vi "VIH HelpGen - Get Control Info.vi"(6 "Ctrl Dscr Params":T5, 8 "error in":errorcluster, 9 "Table Templates":T6, 11 "Ctl Refnum":refnum<vi>) -> (0 "error out":errorcluster, 1 "Image Filename":string, 2 "Ctrl Term Image":T7, 3 "dup Ctl Refnum":refnum<vi>, 4 "Show members":bool, 5 "Ctrl Description":string, 7 "Ctrl Name":string)   [LabVIEW 2014]
doc: "::: VI Helpeks :::\nCopyright (c) 2000-2026 Konstantin Shifershteyn. All rights reserved."
uses:
  <vilib>/picture/picture.llb/imagedata.ctl
  VIH HelpGen Typedef - Table Templates Cluster - VI Help.ctl
  VIH HelpGen Typedef - Cluster - Control Rule.ctl
  VIH HelpGen Typedef - Enum - Description Mode.ctl
  VIH HelpGen Typedef - Enum - Default,Enable,Disable.ctl
  VIH HelpGen Typedef - Cluster - Enum Value Info.ctl
panel:
  # "VI Helpeks\nCopyright (c) 2012-2026 Konstantin Shifershteyn"
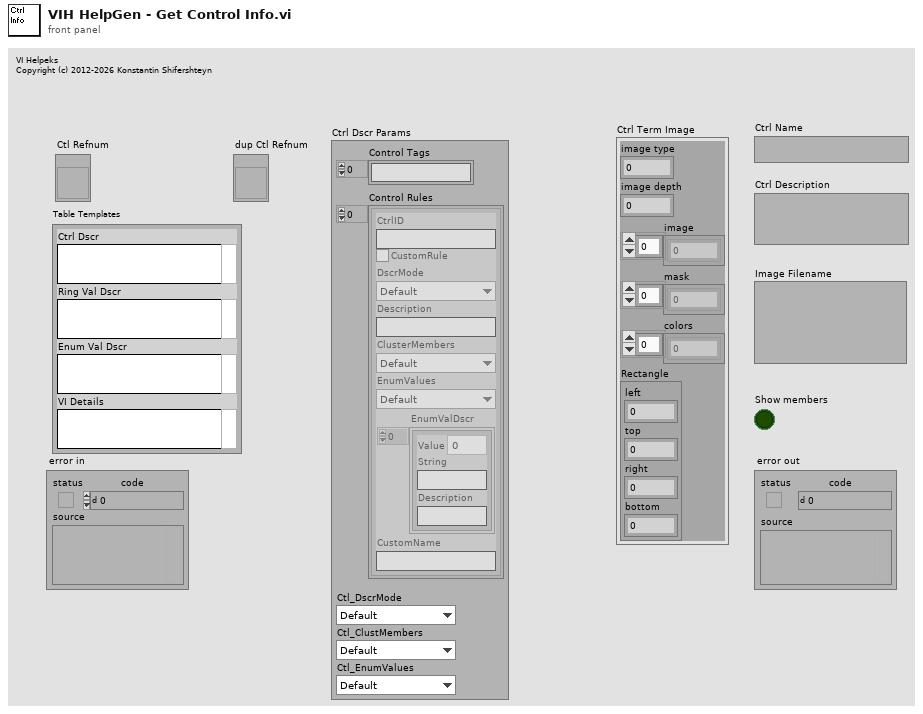
[diagram p1: front panel]
types:
  T1 = typedef "VIH HelpGen Typedef - Cluster - Control Rule.ctl" = cluster{"CtrlID":string, "CustomRule":bool, "DscrMode":T2, "Description":string, "ClusterMembers":T3, "EnumValues":T3, "EnumValDscr":T4[], "CustomName":string}
  T2 = typedef "VIH HelpGen Typedef - Enum - Description Mode.ctl" = enum16{"Default", "Description", "Description1", "Description2", "Custom", "None"}
  T3 = typedef "VIH HelpGen Typedef - Enum - Default,Enable,Disable.ctl" = enum16{"Default", "Enable", "Disable"}
  T4 = typedef "VIH HelpGen Typedef - Cluster - Enum Value Info.ctl" = cluster{"Value":ext, "String":string, "Description":string}
  T5 = cluster{"Control Tags":string[], "Control Rules":T1[], "Ctl_DscrMode":T2, "Ctl_ClustMembers":T3, "Ctl_EnumValues":T3}
  T6 = typedef "VIH HelpGen Typedef - Table Templates Cluster - VI Help.ctl" = cluster{"Ctrl Dscr":string, "Ring Val Dscr":string, "Enum Val Dscr":string, "VI Details":string}
  T7 = typedef "imagedata.ctl" = cluster{"image type":i32, "image depth":i32, "image":u8[], "mask":u8[], "colors":u32[], "Rectangle":cluster{"left":i16, "top":i16, "right":i16, "bottom":i16}}
  T8 = enum32{"not a typedef", "typedef", "strict typedef", "class private data"}
  T9 = enum16{"none", "LV description", "VH minimum", "VH extended"}
  T10 = typedef "LVStringsAndValuesArrayTypeDef.ctl" = cluster{"String":string, "Value":ext}[]
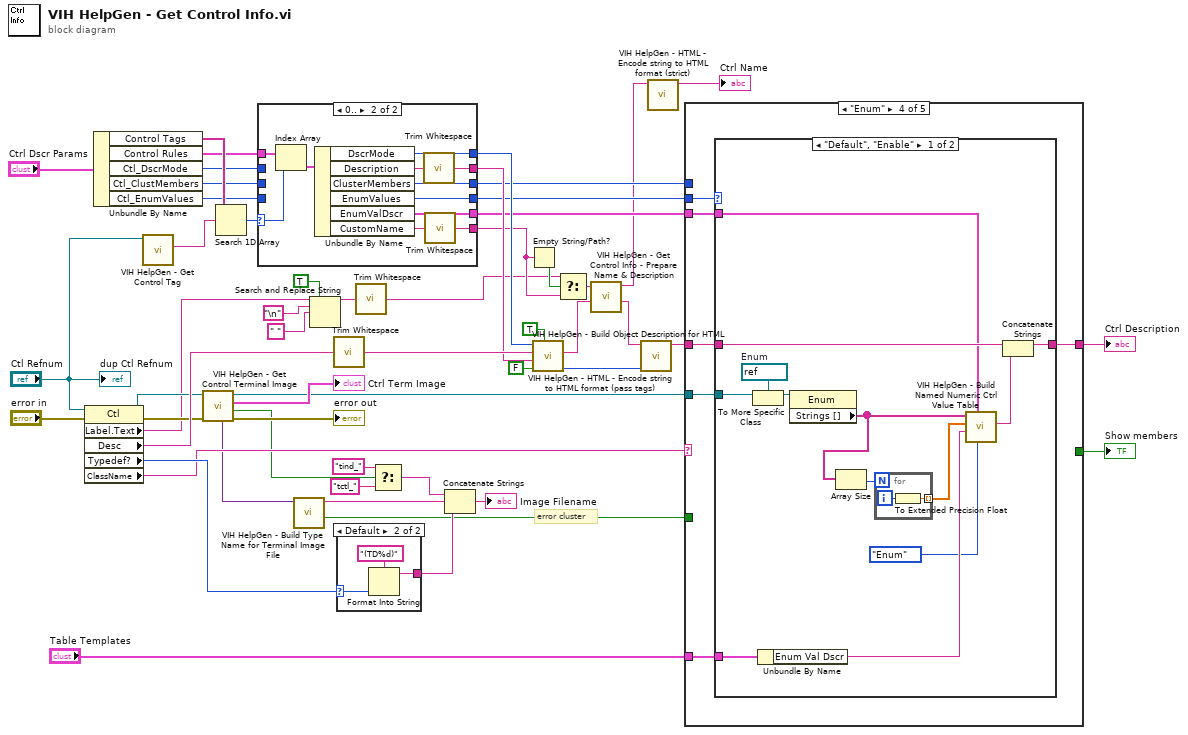
[diagram p0: block diagram]
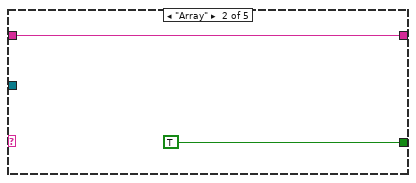
[diagram p4: hidden frame]
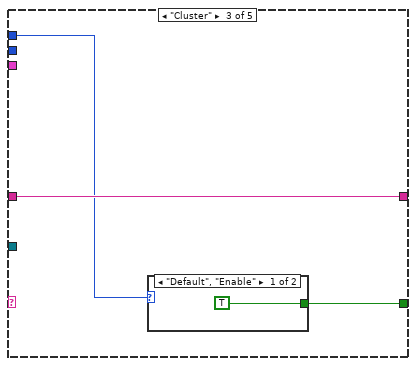
[diagram p5: hidden frame]
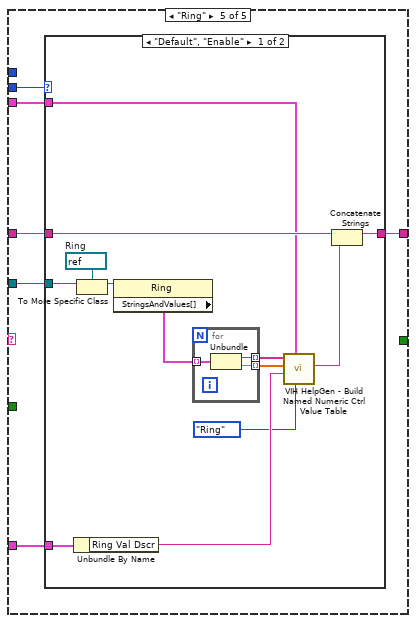
[diagram p8: hidden frame]
diagram:
  # "error cluster"
  n1 = property class="Ctl"(reference="Ctl Refnum", error in="error in") -> (reference out=w50:refnum<vi>, error out=w51:errorcluster, "Label.Text"=w7:string, "Desc"=w53:string, "Typedef?"=w43:T8, "ClassName"=w37:string)
  n2 = Unbundle By Name("Ctrl Dscr Params") -> ("Control Tags"=w31:string[], "Control Rules"=w29:T1[], "Ctl_DscrMode"=w26:T2, "Ctl_ClustMembers"=w27:T3, "Ctl_EnumValues"=w28:T3)
  n3 = call "VIH HelpGen - Get Control Tag.vi"("Ctl Refnum"="Ctl Refnum") -> ("Control Tag"=w18:string)  [unwired: 5 in, 5 out]
  n4 = call "VIH HelpGen - Get Control Terminal Image.vi"("error in"=w51, "Ctl Refnum"=w50) -> ("error out"=→"error out":errorcluster, "Indicator"=w33:bool, "Ctrl Term Icon"=→"Ctrl Term Image":T7, "dup Ctl Refnum"=w36:refnum<vi>, "Data Type"=w34:variant)  [unwired: 5 in]
  n5 = Search 1D Array(1D array=w31, element=w18) -> (index of element=w30:i32)  [unwired: 1 in]
  n6 = case shown="0.." w30 {
    selector: w30 -> [_ w66]
    tunnel: w29 -> [_ w67]
    tunnel: [w56 w64] -> w20
    tunnel: w28 -> [w56 _]
    tunnel: [w55 w63] -> w21
    tunnel: w27 -> [w55 _]
    tunnel: [_ w58] -> w23
    tunnel: [w54 w61] -> w24
    tunnel: w26 -> [w54 _]
    tunnel: [_ w60] -> w15
    tunnel: [_ w57] -> w12
    frame ..-1 {
    }
    frame 0.. {
      n7 = Index Array(array=w67, index=w66) -> (element=w65:T1)
      n8 = Unbundle By Name(w65) -> ("DscrMode"=w61:T2, "Description"=w62:string, "ClusterMembers"=w63:T3, "EnumValues"=w64:T3, "EnumValDscr"=w60:T4[], "CustomName"=w59:string)
      n9 = call <vilib>:"Trim Whitespace.vi"("string"=w62) -> ("trimmed string"=w58:string)  [unwired: 1 in]
      n10 = call <vilib>:"Trim Whitespace.vi"("string"=w59) -> ("trimmed string"=w57:string)  [unwired: 1 in]
    }
  }
  n11 = call "VIH HelpGen - Build Type Name for Terminal Image File.vi"("variant"=w34) -> ("Error Cluster"=w40:bool, "Name"=w44:string)  [unwired: 9 in]
  n12 = Search and Replace String(replace all?=TRUE, input string=w7, search string="\n", replace string=" ") -> (result string=w6:string)  [unwired: 4 in, 3 out]
  n13 = call <vilib>:"Trim Whitespace.vi"("string"=w53) -> ("trimmed string"=w25:string)  [unwired: 1 in]
  n14 = case shown="Default" w43 {
    selector: w43 -> [_ w69]
    tunnel: [_ w68] -> w41
    frame "not a typedef" {
    }
    frame Default {
      n15 = Format Into String(format string="(TD%d)", w69) -> (resulting string=w68:string)  [unwired: 2 in, 1 out]
    }
  }
  n16 = call <vilib>:"Trim Whitespace.vi"("string"=w6) -> ("trimmed string"=w11:string)  [unwired: 1 in]
  n17 = Select(t="tind_", s=w33, f="tctl_") -> (s? t:f=w42:string)
  n18 = Concatenate Strings(w42, w44, w41) -> (→"Image Filename":string)
  n19 = Empty String/Path?(string/path=w12) -> (empty?=w13:bool)
  n20 = call "VIH HelpGen - Build Object Description for HTML.vi"("Ena \"No Description\" message (F)"=TRUE, "Generate \"HTML Description\" (T)"=FALSE ("Generate \"Description HTML\" (T)"), "Custom Description"=w23, "Default Description"=w25, "DscrMode"=w24) -> ("HTML Tagset allowed"=w3:T9, "Description HTML out"=w1:string)  [unwired: 5 in]
  n21 = Select(t=w11, s=w13, f=w12) -> (s? t:f=w14:string)
  n22 = call "VIH HelpGen - Get Control Info - Prepare Name & Description.vi"("Description"=w1, "Name"=w14) -> ("Description out"=w17:string, "Name out"=w5:string)  [unwired: 8 in]
  n23 = call "VIH HelpGen - HTML - Encode string to HTML format (pass tags).vi"("HTML Tagset allowed"=w3, "string"=w17) -> ("HTML string"=w16:string)  [unwired: 9 in]
  n24 = call "VIH HelpGen - HTML - Encode string to HTML format (strict).vi"("string"=w5) -> ("HTML string"=→"Ctrl Name":string)  [unwired: 10 in]
  n25 = case shown="\"Enum\"" w37 {
    tunnel: w40 -> [_ _ _ _ _]
    tunnel: w16 -> [w71 w73 w76 w82 w104]
    tunnel: [w71 w73 w76 w81 w102] -> w39
    tunnel: [_ TRUE w75 _ _] -> w38
    tunnel: w36 -> [_ _ _ w83 w105]
    tunnel: "Table Templates" -> [_ _ _ w80 w103]
    tunnel: w21 -> [_ _ w74 _ _]
    tunnel: w20 -> [_ _ _ w79 w101]
    tunnel: w15 -> [_ _ _ w78 w100]
    frame Default {
    }
    frame "Array" {
    }
    frame "Cluster" {
      n26 = case shown="\"Default\", \"Enable\"" w74 {
        tunnel: [TRUE _] -> w75
        frame "Default", "Enable" {
        }
        frame "Disable" {
        }
      }
    }
    frame "Enum" {
      n27 = case shown="\"Default\", \"Enable\"" w79 {
        tunnel: w83 -> [w96 _]
        tunnel: w82 -> [w93 w99]
        tunnel: [w91 w99] -> w81
        tunnel: w80 -> [w88 _]
        tunnel: w78 -> [w85 _]
        frame "Default", "Enable" {
          w95 = refnum<vi> refnum  # Enum
          n28 = To More Specific Class(target class=w95, reference=w96) -> (specific class reference=w94:refnum<vi>)  [unwired: 1 in, 1 out]
          n29 = Unbundle By Name(w88) -> ("Enum Val Dscr"=w87:string)
          n30 = property class="Enum"(reference=w94) -> ("Strings []"=w86:string[])  [unwired: 1 in, 2 out]
          n31 = Array Size(array=w86) -> (size(s)=w92:i32)
          n32 = for {
            N: w92 -> [_]
            tunnel: [w97] -> w90 mode=indexing
            i -> [w98]
            n33 = To Extended Precision Float(1:w98) -> (0:w97:ext)
          }
          n34 = call "VIH HelpGen - Build Named Numeric Ctrl Value Table.vi"("Class"=enum16{"Enum", "Ring"}."Enum", "EnumValDscr"=w85, "Table Template"=w87, "Values"=w90, "Names"=w86) -> ("HTML out"=w89:string)  [unwired: 6 in]
          n35 = Concatenate Strings(w93, w89) -> (w91:string)
        }
        frame "Disable" {
        }
      }
    }
    frame "Ring" {
      n36 = case shown="\"Default\", \"Enable\"" w101 {
        tunnel: w105 -> [w118 _]
        tunnel: w104 -> [w115 w122]
        tunnel: w103 -> [w111 _]
        tunnel: [w109 w122] -> w102
        tunnel: w100 -> [w107 _]
        frame "Default", "Enable" {
          w117 = refnum<vi> refnum  # Ring
          n37 = Unbundle By Name(w111) -> ("Ring Val Dscr"=w110:string)
          n38 = To More Specific Class(target class=w117, reference=w118) -> (specific class reference=w116:refnum<vi>)  [unwired: 1 in, 1 out]
          n39 = property class="Ring"(reference=w116) -> ("StringsAndValues[]"=w114:T10)  [unwired: 1 in, 2 out]
          n40 = for {
            tunnel: w114 -> [w121] mode=indexing
            tunnel: [w120] -> w113 mode=indexing
            tunnel: [w119] -> w112 mode=indexing
            n41 = Unbundle(w121) -> ("String"=w120:string, "Value"=w119:ext)
          }
          n42 = call "VIH HelpGen - Build Named Numeric Ctrl Value Table.vi"("Class"=enum16{"Enum", "Ring"}."Ring", "EnumValDscr"=w107, "Table Template"=w110, "Values"=w112, "Names"=w113) -> ("HTML out"=w108:string)  [unwired: 6 in]
          n43 = Concatenate Strings(w115, w108) -> (w109:string)
        }
        frame "Disable" {
        }
      }
    }
  }
  "Ctrl Description" <- w39
  "Show members" <- w38
  "dup Ctl Refnum" <- "Ctl Refnum"
